vi "VIH ProjFile - File Tree - Write.vi"(4 "Tree Parent Tag":string, 6 "Project Tree":T1, 8 "error in":errorcluster, 10 "Project Folder":path, 11 "XML Parent Item":refnum<k20>) -> (0 "error out":errorcluster, 3 "dup XML Parent Item":refnum<k20>)   [LabVIEW 2014]
doc: "::: VI Helpeks :::\nCopyright (c) 2000-2026 Konstantin Shifershteyn. All rights reserved."
uses:
  _VIH Project Manager.llb/VIH Project Tree Typedef - Tree Refnum.ctl
  <vilib>/xml/Close Reference(Node).vi
  <resource>/objmgr/DOMUserDefRef.rc
  <vilib>/xml/NI_XML.lvlib
panel:
  # "VI Helpeks\nCopyright (c) 2012-2026 Konstantin Shifershteyn"
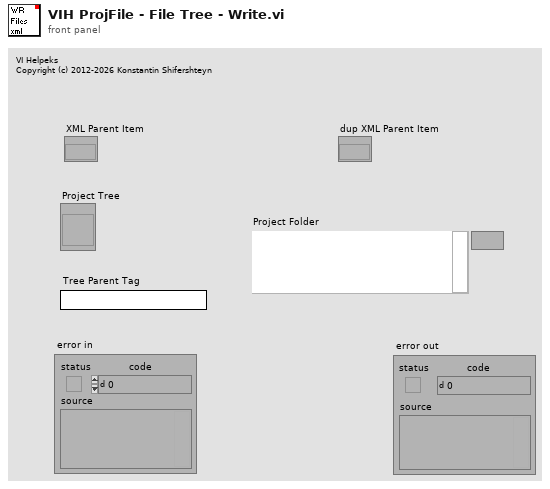
[diagram p1: front panel]
types:
  T1 = typedef "VIH Project Tree Typedef - Tree Refnum.ctl" = refnum<vi>
  T2 = typedef "VIH Project Tree Typedef - Tree Item Type.ctl" = enum32{"<Invalid>", "Project", "Proj Files", "Proj Rules", "File Group", "Rule Group", "Any File", "LV Func", ".mnu", ".mnu (dyn)", ".vi", ".vi (dyn)", ".vit", ".vit (dyn)", ".ctl", ".ctl (dyn)", ".ctt", ".ctt (dyn)", "polyVI", "polyVI (dyn)", "expVI", "expVI (dyn)", "HTML", "PolyVI Inst"}
  T3 = typedef "VIH HelpGen Typedef - Cluster - Group Rule.ctl" = cluster{"Source Root Dir":path, "Build Root Dir":path, "BuildHelp":T4, "Source Paths":T5, "Target Paths":T6, "VIDscrMode":T7, "MenuDscrMode":T7, "MenuItemIcons":T4, "Control Rules":T8[], "Flags":T10, "Ctl_DscrMode":T7, "Ctl_ClustMembers":T4, "Ctl_EnumValues":T4, "%Comments":string, "PVIIDscrMode":T7, "VIDetailsMode":T7, "ProductInfoMode":T4, "ProductInfoText":string}
  T4 = typedef "VIH HelpGen Typedef - Enum - Default,Enable,Disable.ctl" = enum16{"Default", "Enable", "Disable"}
  T5 = typedef "VIH HelpGen Typedef - Cluster - Group Rule - Source Paths.ctl" = cluster{"CSS Files":path[], "JS Files":path[], "VI Template":path, "Menu Template":path, "PolyVI Template":path}
  T6 = typedef "VIH HelpGen Typedef - Cluster - Group Rule - Target Paths.ctl" = cluster{"HTML Dir":path, "Image Dir":path, "CSS Dir":path, "JS Dir":path}
  T7 = typedef "VIH HelpGen Typedef - Enum - Description Mode.ctl" = enum16{"Default", "Description", "Description1", "Description2", "Custom", "None"}
  T8 = typedef "VIH HelpGen Typedef - Cluster - Control Rule.ctl" = cluster{"CtrlID":string, "CustomRule":bool, "DscrMode":T7, "Description":string, "ClusterMembers":T4, "EnumValues":T4, "EnumValDscr":T9[], "CustomName":string}
  T9 = typedef "VIH HelpGen Typedef - Cluster - Enum Value Info.ctl" = cluster{"Value":ext, "String":string, "Description":string}
  T10 = typedef "VIH HelpGen Typedef - Cluster - Group Rule - Flags.ctl" = cluster{"Override CSS Files":bool, "Override JS Files":bool, "Override Ctl Rules":bool}
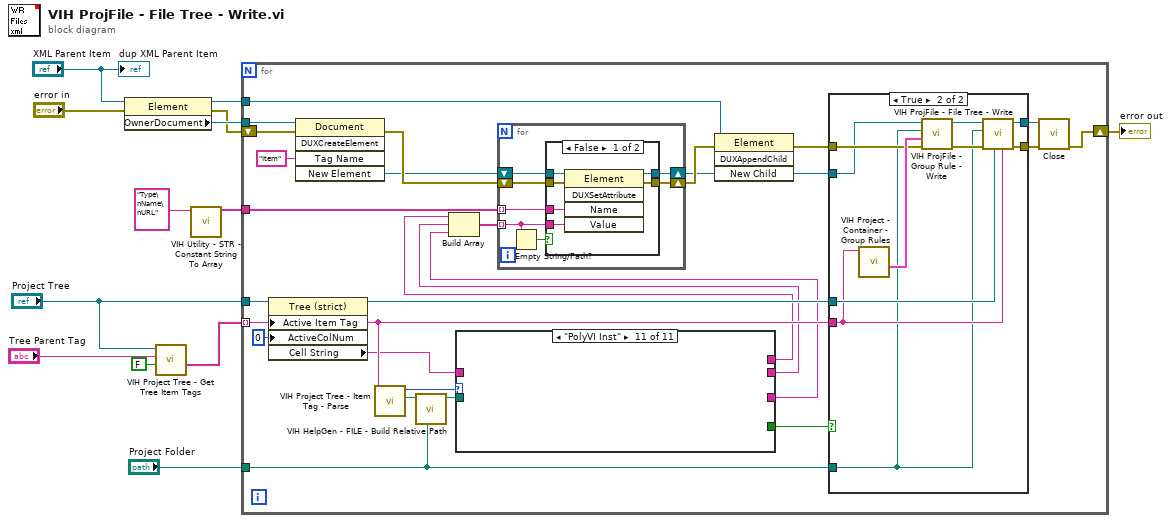
[diagram p0: block diagram]
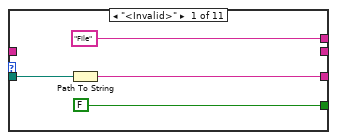
[diagram p2: hidden frame]
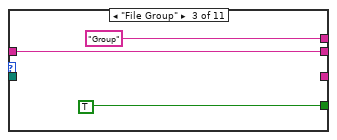
[diagram p4: hidden frame]
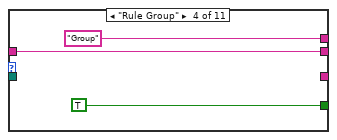
[diagram p5: hidden frame]
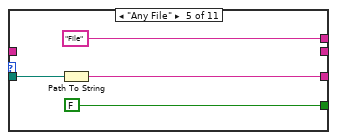
[diagram p6: hidden frame]
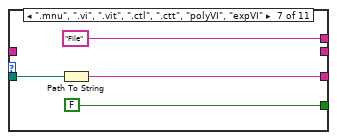
[diagram p8: hidden frame]
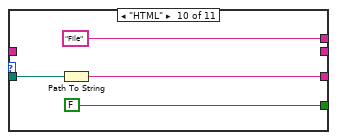
[diagram p11: hidden frame]
diagram:
  n1 = property class="Element"(reference="XML Parent Item", error in="error in") -> (reference out=w8:refnum<k20>, error out=w7:errorcluster, "OwnerDocument"=w9:refnum<k20>)
  n2 = call "VIH Project Tree - Get Tree Item Tags.vi"("Recursively (T)"=FALSE, "Parent Item Tag"="Tree Parent Tag", "Project Tree"="Project Tree") -> ("Child Item Tags"=w12:string[])  [unwired: 5 in, 3 out]
  n3 = call "VIH Utility - STR - Constant String To Array.vi"("String in"="Type\nName\nURL") -> ("Array out"=w4:string[])  [unwired: 10 in]
  n4 = for {
    tunnel: w9 -> [w40]
    shift-right: [w33] -> w11
    shift-left: w7 -> [w39]
    tunnel: w8 -> [w34]
    tunnel: "Project Tree" -> [w37]
    tunnel: w12 -> [w23] mode=indexing
    tunnel: w4 -> [w25]
    tunnel: "Project Folder" -> [w18]
    n5 = property class="Tree (strict)"(reference=w37, "Active Item Tag"=w23, "ActiveColNum"=0 ("Active Cell:Active Column Number")) -> (reference out=w32:T1, "Cell String"=w15:string)  [unwired: 1 in, 1 out]
    n6 = invoke class="Document" method="DUXCreateElement"(reference=w40, error in=w39, "Tag Name"="Item") -> (error out=w27:errorcluster, "New Element"=w26:refnum<k20>)  [unwired: 2 in, 3 out]
    n7 = call "VIH Project Tree - Item Tag - Parse.vi"("Tree Item Tag"=w23) -> ("Item File Path"=w20:path, "Item Type"=w22:T2)  [unwired: 8 in, 1 out]
    n8 = call "VIH HelpGen - FILE - Build Relative Path.vi"("Root Path"=w18, "Path in"=w20) -> ("Path out"=w19:path)  [unwired: 9 in]
    n9 = case shown="\"PolyVI Inst\"" w22 {
      tunnel: ["File" _ "Group" "Group" "File" _ "File" _ _ "File" _] -> w16
      tunnel: [FALSE _ TRUE TRUE FALSE _ FALSE _ _ FALSE _] -> w21
      tunnel: [w43 _ _ _ w51 _ w55 _ _ w59 _] -> w17
      tunnel: w19 -> [w44 _ _ _ w52 _ w56 _ _ w60 _]
      tunnel: [_ _ w45 w48 _ _ _ _ _ _ _] -> w14
      tunnel: w15 -> [_ _ w45 w48 _ _ _ _ _ _ _]
      frame "<Invalid>" {
        n10 = Path To String(path=w44) -> (string=w43:string)
      }
      frame "Project".."Proj Rules" {
      }
      frame "File Group" {
      }
      frame "Rule Group" {
      }
      frame "Any File" {
        n11 = Path To String(path=w52) -> (string=w51:string)
      }
      frame "LV Func" {
      }
      frame ".mnu", ".vi", ".vit", ".ctl", ".ctt", "polyVI", "expVI" {
        n12 = Path To String(path=w56) -> (string=w55:string)
      }
      frame ".mnu (dyn)", ".vi (dyn)", ".vit (dyn)" {
      }
      frame ".ctl (dyn)", ".ctt (dyn)", "polyVI (dyn)", "expVI (dyn)" {
      }
      frame "HTML" {
        n13 = Path To String(path=w60) -> (string=w59:string)
      }
      frame "PolyVI Inst" {
      }
    }
    n14 = Build Array(w16, w14, w17) -> (w24:string[])
    n15 = for {
      tunnel: w24 -> [w63] mode=indexing
      shift-right: [w69] -> w35
      shift-left: w27 -> [w66]
      shift-right: [w68] -> w29
      shift-left: w26 -> [w67]
      tunnel: w25 -> [w65] mode=indexing
      n16 = Empty String/Path?(string/path=w63) -> (empty?=w64:bool)
      n17 = case shown="False" w64 {
        tunnel: [w75 w76] -> w69
        tunnel: w63 -> [w74 _]
        tunnel: [w73 w77] -> w68
        tunnel: w67 -> [w72 w77]
        tunnel: w66 -> [w71 w76]
        tunnel: w65 -> [w70 _]
        frame False {
          n18 = invoke class="Element" method="DUXSetAttribute"(reference=w72, error in=w71, "Name"=w70, "Value"=w74) -> (reference out=w73:refnum<k20>, error out=w75:errorcluster)  [unwired: 1 in, 3 out]
        }
        frame True {
        }
      }
    }
    n19 = invoke class="Element" method="DUXAppendChild"(reference=w34, error in=w35, "New Child"=w29) -> (error out=w28:errorcluster)  [unwired: 1 in, 3 out]
    n20 = case shown="True" w21 {
      tunnel: w28 -> [w79 w83]
      tunnel: w29 -> [w78 w81]
      tunnel: w32 -> [_ w89]
      tunnel: [w79 w88] -> w31
      tunnel: [w78 w82] -> w30
      tunnel: w23 -> [_ w87]
      tunnel: w18 -> [_ w80]
      frame False {
      }
      frame True {
        n21 = call "VIH Project - Container - Group Rules.vi"("Group ID"=w87) -> ("Group Rule out"=w86:T3)  [unwired: 6 in, 4 out]
        n22 = call "VIH ProjFile - Group Rule - Write.vi"("error in"=w83, "Group Rule"=w86, "Project Folder"=w80, "XML Parent Item"=w81) -> ("error out"=w84:errorcluster, "dup XML Parent Item"=w85:refnum<k20>)  [unwired: 6 in]
        n23 = call "VIH ProjFile - File Tree - Write.vi"("Tree Parent Tag"=w87, "Project Tree"=w89, "error in"=w84, "Project Folder"=w80, "XML Parent Item"=w85) -> ("error out"=w88:errorcluster, "dup XML Parent Item"=w82:refnum<k20>)  [unwired: 5 in]
      }
    }
    n24 = call-poly <vilib>:"Close.vi"("error in (no error)"=w31, "node"=w30) -> ("error out"=w33:errorcluster)  [unwired: 7 in]
  }
  "error out" <- w11
  "dup XML Parent Item" <- "XML Parent Item"
